vi "周围地雷个数.vi"(1 "索引":i32) -> (0 "数值":i32)   [LabVIEW 2017]
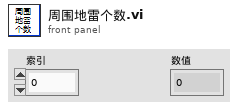
[diagram p1: front panel]
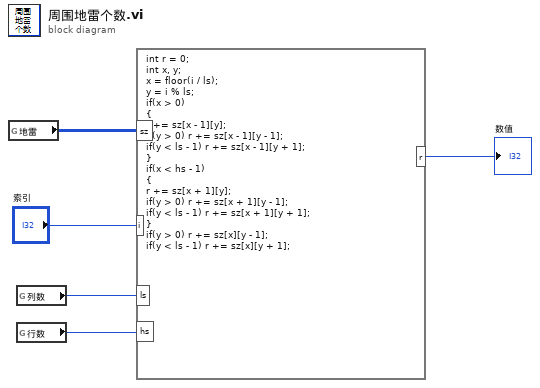
[diagram p0: block diagram]
diagram:
  n1 = global read "全局变量.vi" "地雷"() -> (w3:i16[][])
  n2 = global read "全局变量.vi" "列数"() -> (w2:i32)
  n3 = global read "全局变量.vi" "行数"() -> (w1:i32)
  n4 = formula code="int r = 0;\nint x, y;\nx = floor(i / ls);\ny = i % ls;\nif(x > 0)\n{\nr += sz[x - 1][y];\nif(y > 0) r += sz[x - 1][y - 1];\nif(y < ls - 1) r += sz[x - 1][y + 1];\n}\nif(x < hs - 1)\n{\nr += sz[x + 1][y];\nif(y > 0) r += sz[x + 1][y - 1];\nif(y < ls - 1) r += sz[x + 1][y + 1];\n}\nif(y > 0) r += sz[x][y - 1];\nif(y < ls - 1) r += sz[x][y + 1];"("sz"=w3, "i"="索引", "ls"=w2, "hs"=w1) -> ("r"=→"数值":i32)
